vi "call include vi script.vi"(8 "error in":errorcluster, 11 "state cluster":T1) -> (0 "error out":errorcluster)   [LabVIEW 2014, in "Standard Editor.lvlib"]
uses:
  Standard Editor.lvlib
  Controls/StateCluster.ctl
  Configuration Editor/Classes/SystemConfigRepo/SystemConfigRepo.lvclass
  Configuration Editor/Classes/Systems/Systems.lvclass
  <vilib>/NI/Configuration Framework/Node/StandardEvents.ctl
  <vilib>/NI/Configuration Framework/Node/UserEventRef.ctl
  <vilib>/NI/Configuration Framework/Controls/EventCluster.ctl
  <vilib>/NI/Configuration Framework/Node/NodeChangeEvent.ctl
  <vilib>/NI/Configuration Framework/Node/NodeRef.ctl
  <vilib>/NI/Configuration Framework/Node/NISE_CEF_Node.lvclass
  <vilib>/NI/Configuration Framework/Node/CacheState.ctl
  <vilib>/NI/Configuration Framework/Node/RefreshUIEvent.ctl
  <vilib>/NI/Configuration Framework/Node/StopEvent.ctl
  <vilib>/NI/Configuration Framework/glyph manager/glyph manager.ctl
  <vilib>/picture/picture.llb/imagedata.ctl
  <vilib>/NI/AMC/Message Queue.ctl
  <vilib>/NI/AMC/Message.ctl
  <vilib>/NI/Tools/Keyed Array/KeyedArray.ctl
  Framework Configuration Classes/class cache/PL_class cache.lvlib
  <vilib>/NI/Configuration Framework/tree serializer/NISE_CEF_TreeSerializer.lvlib
  <vilib>/NI/Configuration Framework/NISE_CEF_TreeControl.lvlib
  <vilib>/NI/Configuration Framework/glyph manager/glyph manager.lvlib
  <vilib>/NI/Tools/Keyed Array/Tools_KeyedArray.lvlib
  <vilib>/NI/AMC/AMC.lvlib
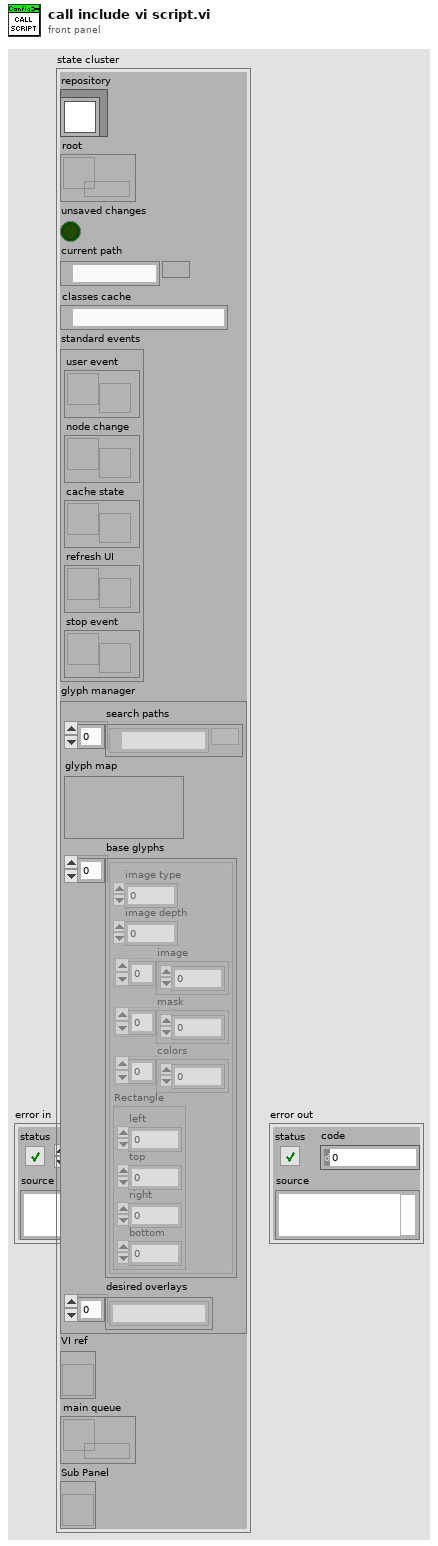
[diagram p1: front panel]
types:
  T1 = typedef "Standard Editor.lvlib/StateCluster.ctl" = cluster{"repository":refnum<class "SystemConfigRepo.lvclass">, "root":refnum<data-value>, "unsaved changes":bool, "current path":path, "classes cache":path, "standard events":T2, "glyph manager":T8, "VI ref":refnum<vi>, "main queue":T10, "Sub Panel":refnum<vi>}
  T2 = typedef "NISE_CEF_Node.lvclass/StandardEvents.ctl" = cluster{"user event":T3, "node change":T4, "cache state":T5, "refresh UI":T6, "stop event":T7}
  T3 = typedef "NISE_CEF_Node.lvclass/UserEventRef.ctl" = refnum<user-event>
  T4 = typedef "NISE_CEF_Node.lvclass/NodeChangeEvent.ctl" = refnum<user-event>
  T5 = typedef "NISE_CEF_Node.lvclass/CacheState.ctl" = refnum<user-event>
  T6 = typedef "NISE_CEF_Node.lvclass/RefreshUIEvent.ctl" = refnum<user-event>
  T7 = typedef "NISE_CEF_Node.lvclass/StopEvent.ctl" = refnum<user-event>
  T8 = typedef "glyph manager.lvlib/glyph manager.ctl" = cluster{"search paths":path[], "glyph map":variant, "base glyphs":T9[], "desired overlays":string[]}
  T9 = typedef "imagedata.ctl" = cluster{"image type":i32, "image depth":i32, "image":u8[], "mask":u8[], "colors":u32[], "Rectangle":cluster{"left":i16, "top":i16, "right":i16, "bottom":i16}}
  T10 = typedef "AMC.lvlib/Message Queue.ctl" = refnum<queue>
  T11 = typedef "PL_class cache.lvlib/cache definition.ctl" = cluster{"configuration":T12, "class cache data":T13}
  T12 = typedef "PL_class cache.lvlib/cache search configuration.ctl" = cluster{"Search Paths":path[], "Folders to Exclude":string[], "full class list":path[]}
  T13 = typedef "PL_class cache.lvlib/cached class information.ctl" = cluster{"targets":T14[], "engines":T15[], "modules":T15[], "ignored class list":path[]}
  T14 = typedef "PL_class cache.lvlib/target class metadata.ctl" = cluster{"file name":string, "fully qualified name":string, "menu display name":string, "configuration class name":string}
  T15 = typedef "PL_class cache.lvlib/class metadata.ctl" = cluster{"file name":string, "fully qualified name":string, "menu display name":string, "configuration class":string, "category":string, "instances allowed":i32, "supported targets":T16[]}
  T16 = typedef "TBM configuration.lvclass/Target Types.ctl" = enum16{"Windows", "Mac", "Linux", "Linux RT ARM", "VxWorks", "Pharlap", "Other", "Linux RT x64"}
  T17 = typedef "NISE_CEF_TreeSerializer.lvlib/base file format.ctl" = cluster{"version":string, "data":string}
  T18 = typedef "NISE_CEF_TreeSerializer.lvlib/flat hierarchy.ctl" = cluster{"hierarchy structure":T19, "instance data":T21[]}
  T19 = typedef "NISE_CEF_TreeSerializer.lvlib/full hierarchy.ctl" = cluster{"root":string, "hierarchy":T20[]}
  T20 = typedef "NISE_CEF_TreeSerializer.lvlib/hierarchy element.ctl" = cluster{"current node":string, "children":string[]}
  T21 = typedef "NISE_CEF_TreeSerializer.lvlib/instance data.ctl" = cluster{"ID":string, "Alias":string, "class":string, "version":string, "data":string}
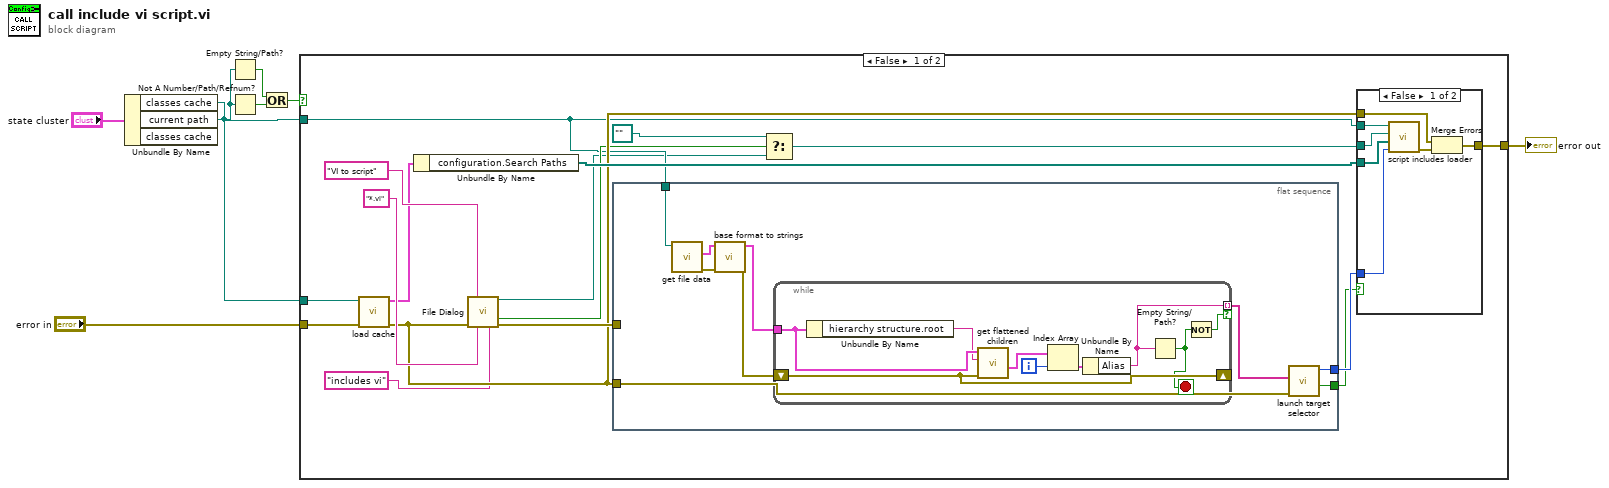
[diagram p0: block diagram]
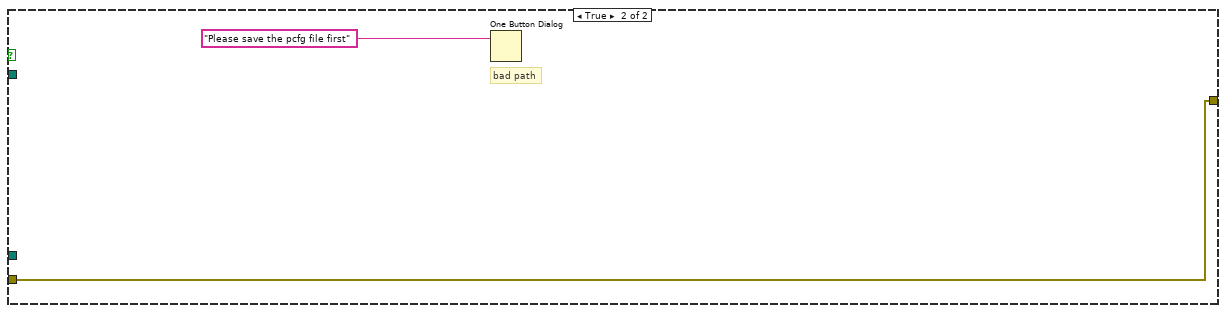
[diagram p3: hidden frame]
diagram:
  n1 = Unbundle By Name("state cluster") -> ("classes cache"=w6:path, "current path"=w5:path)  [unwired: 1 out]
  n2 = Empty String/Path?(string/path=w5) -> (empty?=w3:bool)
  n3 = Not A Number/Path/Refnum?(number/path/refnum=w5) -> (NaN/Path/Refnum?=w2:bool)
  n4 = Or(x=w3, y=w2) -> (x .or. y?=w4:bool)
  n5 = case shown="False" w4 {
    tunnel: w5 -> [w10 _]
    tunnel: w6 -> [w21 _]
    tunnel: "error in" -> [w20 w52]
    tunnel: [w19 w52] -> w8
    frame False {
      n6 = call "load cache.vi"("error in"=w20, "cache path"=w21) -> ("error out"=w17:errorcluster, "cache"=w23:T11)  [unwired: 8 in]
      n7 = Unbundle By Name(w23) -> ("configuration.Search Paths"=w22:path[])
      n8 = call "File Dialog"("prompt"="VI to script", "error in"=w17, "pattern (all files)"="*.vi", "pattern label"="includes vi") -> ("selected path"=w9:path, "cancelled"=w15:bool, "error out"=w18:errorcluster)  [unwired: 8 in, 1 out]
      n9 = flat-sequence {
        tunnel: [w41] -> w14
        tunnel: w18 -> [_]
        tunnel: w17 -> [w42]
        tunnel: [w40] -> w11
        tunnel: w10 -> [w37]
        frame #0 {
          n10 = call <vilib>:"get file data.vi"("Path"=w37) -> ("error out"=w38:errorcluster, "format"=w39:T17)  [unwired: 9 in]
          n11 = call <vilib>:"base format to strings.vi"("error in"=w38, "format"=w39) -> ("error out"=w36:errorcluster, "data"=w35:T18)  [unwired: 8 in]
          n12 = while {
            shift-right: [w46] -> _
            shift-left: w36 -> [w46]
            tunnel: w35 -> [w49]
            tunnel: [w45] -> w34 mode=indexing if=w44
            i -> [w47]
            stop <- w43 stop-if-true
            n13 = Unbundle By Name(w49) -> ("hierarchy structure.root"=w48:string)
            n14 = call <vilib>:"get flattened children.vi"("error in"=w46, "ID"=w48, "flat hierarchy"=w49) -> ("children"=w51:T21[])  [unwired: 7 in, 1 out]
            n15 = Index Array(array=w51, index=w47) -> (element=w50:T21)
            n16 = Unbundle By Name(w50) -> ("Alias"=w45:string)
            n17 = Empty String/Path?(string/path=w45) -> (empty?=w43:bool)
            n18 = Not(x=w43) -> (.not. x?=w44:bool)
          }
          n19 = call "launch target selector.vi"("error in (no error)"=w42, "Options"=w34) -> ("Canceled?"=w40:bool, "Target Index"=w41:i32)  [unwired: 7 in, 1 out]
        }
      }
      n20 = Select(t=path "", s=w15, f=w9) -> (s? t:f=w13:path)
      n21 = case shown="False" w11 {
        tunnel: w10 -> [w32 _]
        tunnel: w22 -> [w31 _]
        tunnel: w14 -> [w30 _]
        tunnel: [w28 w33] -> w19
        tunnel: w17 -> [w27 w33]
        tunnel: w13 -> [w26 _]
        frame False {
          n22 = call "script includes loader.vi"("target"=w30, "Plugin Search Paths"=w31, "vi path (blank=new)"=w26, "pcfg file path"=w32) -> ("error out"=w29:errorcluster)  [unwired: 7 in]
          n23 = Merge Errors(w27, w29) -> (w28:errorcluster)
        }
        frame True {
        }
      }
    }
    frame True {
      # "bad path"
      n24 = One Button Dialog(message="Please save the pcfg file first") -> ()  [unwired: 1 in, 1 out]
    }
  }
  "error out" <- w8
